vi "Test Read Day Entries DST.vi"(8 "error in (no error)":errorcluster, 10 "Work Folder":path, 11 "Test Data Folder":path) -> (0 "error out":errorcluster, 2 "Report":string, 3 "Passed":bool)   [LabVIEW 2026]
doc: "Checks that Read Day Entries returns the entries of one LOCAL day across the daylight saving changes. The cases assume the PC runs in US Central time (CST/CDT): Sun 8 Mar 2026 is a 23-hour day and Sun 1 Nov 2026 a 25-hour day. Six 30-minute entries are saved with Time Entry Store-INI: A at 23:30 CDT on 8 Mar, B at 00:30 CDT on 9 Mar, C at 23:30 CST on 1 Nov, D at 00:30 CST on 2 Nov, E at 00:30 CDT on 1 Nov and F at 23:30 CST on 7 Mar. Read Day Entries is then called for local noon of 8 Mar, 9 Mar, 1 Nov and 2 Nov: the entry count of each day is checked (1, 1, 2, 1), then that each expected entry ID is among the returned IDs (8 Mar: A, 9 Mar: B, 1 Nov: E and C, 2 Nov: D), independent of order - 9 checks.\n\nInputs: Test Data Folder holds the source copies (Samples); each run works in a new case folder (read-day-dst) under Work Folder. Passed is TRUE when every check passed and no error occurred; Report lists every check.\n\nGenerated by: Claude"
uses:
  Storage/Project Store-INI/Project Store-INI.lvclass
  Storage/Time Entry Store-INI/Time Entry Store-INI.lvclass
  Utilities/Time Management/Time Management.lvlib
  Storage/Time Entry Store/Time Entry Store.lvclass
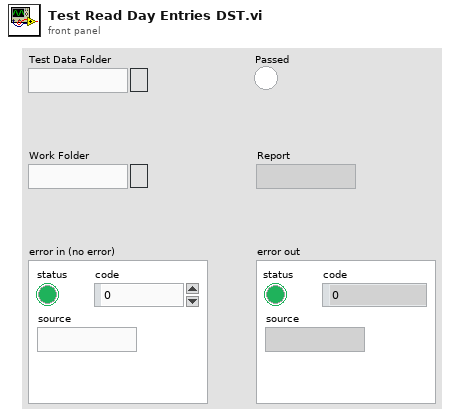
[diagram p1: front panel]
types:
  T1 = cluster{"ID":string, "Project ID":string, "Task ID":string, "Start Time":timestamp, "End Time":timestamp, "Description":string}
  T2 = typedef "Time Entry.ctl" = cluster{"ID":string, "Project ID":string, "Task ID":string, "Start Time":timestamp, "End Time":timestamp, "Description":string}
  T3 = cluster{"ID":string, "Project ID":string, "Task ID":string, "Start Time":timestamp, "End Time":timestamp, "Description":string}[]
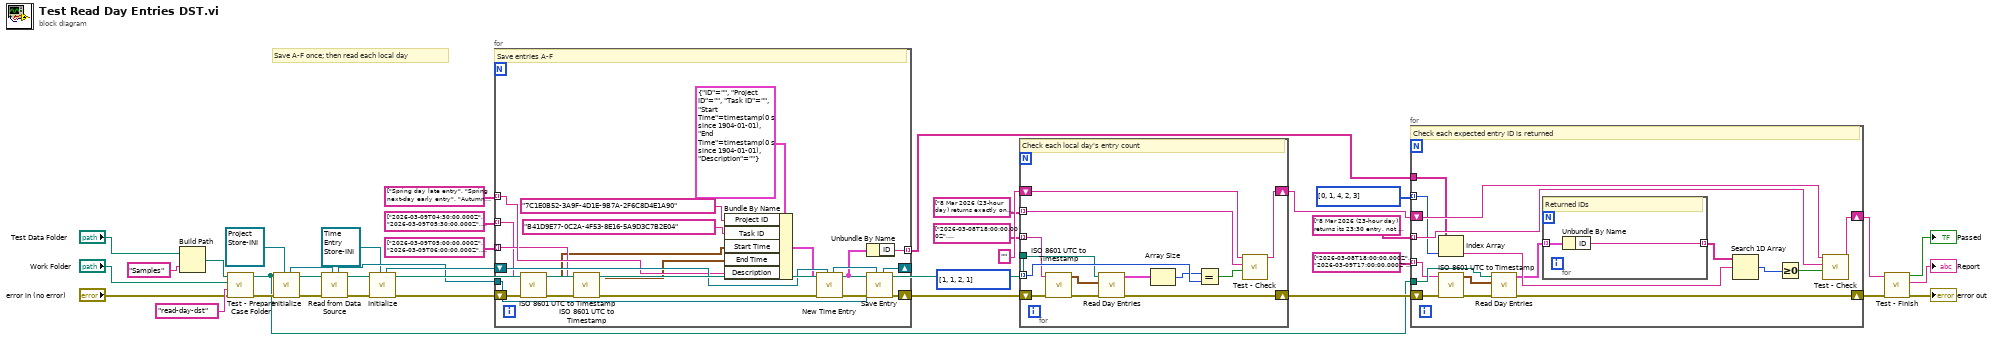
[diagram p0: block diagram]
diagram:
  # "Save A-F once; then read each local day"
  n1 = Build Path(base path="Test Data Folder", name or relative path="Samples" ("Samples")) -> (appended path=w31:path)
  n2 = call "Test - Prepare Case Folder.vi"("error in (no error)"="error in (no error)", "Case Name"="read-day-dst", "Work Folder"="Work Folder", "Source Folder"=w31) -> ("error out"=w32:errorcluster, "Case Folder"=w26:path)  [unwired: 6 in]
  n3 = call-dynamic "Initialize.vi"("Project Store in"=refnum<class "Project Store-INI.lvclass"> refnum ("Project Store-INI"), "error in (no error)"=w32, "Data Folder"=w26) -> ("error out"=w33:errorcluster, "Project Store out"=w34:refnum<class "Project Store-INI.lvclass">)  [unwired: 7 in]
  n4 = call-dynamic "Read from Data Source.vi"("Project Store in"=w34, "error in (no error)"=w33) -> ("error out"=w35:errorcluster, "Project Store out"=w21:refnum<class "Project Store-INI.lvclass">)  [unwired: 8 in]
  n5 = call-dynamic "Initialize.vi"("Time Entry Store in"=refnum<class "Time Entry Store-INI.lvclass"> refnum ("Time Entry Store-INI"), "error in (no error)"=w35, "Data Folder"=w26) -> ("error out"=w23:errorcluster, "Time Entry Store out"=w25:refnum<class "Time Entry Store-INI.lvclass">)  [unwired: 7 in]
  n6 = for {
    tunnel: string[] ["2026-03-09T04:30:00.000Z", "2026-03-09T05:30:00.000Z", "2026-11-02T05:30:00.000Z", "2026-11-02T06:30:00.000Z", "2026-11-01T05:30:00.000Z", "2026-03-08T05:30:00.000Z"] ("Start Times") -> [w42] mode=indexing
    tunnel: string[] ["2026-03-09T05:00:00.000Z", "2026-03-09T06:00:00.000Z", "2026-11-02T06:00:00.000Z", "2026-11-02T07:00:00.000Z", "2026-11-01T06:00:00.000Z", "2026-03-08T06:00:00.000Z"] ("End Times") -> [w45] mode=indexing
    tunnel: string[] ["Spring day late entry", "Spring next-day early entry", "Autumn day late entry", "Autumn next-day early entry", "Autumn day early entry", "Spring previous-day late entry"] ("Descriptions") -> [w47] mode=indexing
    tunnel: w21 -> [w55]
    shift-right: [w53] -> w24
    shift-left: w23 -> [w41]
    shift-right: [w54] -> _
    shift-left: w25 -> [w51]
    tunnel: [w52] -> w22 mode=indexing
    # "Save entries A-F"
    n7 = call "ISO 8601 UTC to Timestamp.vi"("error in (no error)"=w41, "ISO 8601 UTC"=w42) -> ("error out"=w39:errorcluster, "Timestamp"=w40:timestamp)  [unwired: 8 in]
    n8 = call "ISO 8601 UTC to Timestamp.vi"("error in (no error)"=w39, "ISO 8601 UTC"=w45) -> ("error out"=w43:errorcluster, "Timestamp"=w44:timestamp)  [unwired: 8 in]
    n9 = Bundle By Name(cluster=T1 {"ID"="", "Project ID"="", "Task ID"="", "Start Time"=timestamp(0 s since 1904-01-01), "End Time"=timestamp(0 s since 1904-01-01), "Description"=""} ("Time Entry"), "Project ID"="7C1E0B52-3A9F-4D1E-9B7A-2F6C8D4E1A90", "Task ID"="B41D9E77-0C2A-4F53-8E16-5A9D3C7B2E04", "Start Time"=w40, "End Time"=w44, "Description"=w47) -> (w46:T1)
    n10 = call "New Time Entry.vi"("Time Entry Store in"=w51, "error in (no error)"=w43, "Time Entry"=w46) -> ("error out"=w48:errorcluster, "New Time Entry"=w49:T2, "Time Entry Store out"=w50:refnum<class "Time Entry Store-INI.lvclass">)  [unwired: 6 in]
    n11 = Unbundle By Name(w49) -> ("ID"=w52:string)
    n12 = call-dynamic "Save Entry.vi"("Time Entry Store in"=w50, "error in (no error)"=w48, "Project Store"=w55, "Time Entry"=w49) -> ("error out"=w53:errorcluster, "Time Entry Store out"=w54:refnum<class "Time Entry Store-INI.lvclass">)  [unwired: 6 in]
  }
  n13 = for {
    tunnel: string[] ["2026-03-08T18:00:00.000Z", "2026-03-09T17:00:00.000Z", "2026-11-01T18:00:00.000Z", "2026-11-02T18:00:00.000Z"] ("Dates") -> [w59] mode=indexing
    tunnel: string[] ["8 Mar 2026 (23-hour day) returns exactly one entry", "9 Mar 2026 returns exactly one entry", "1 Nov 2026 (25-hour day) returns 2 entries", "2 Nov 2026 returns exactly one entry"] ("Count Check Names") -> [w67] mode=indexing
    tunnel: i32[] [1, 1, 2, 1] ("Expected Counts") -> [w65] mode=indexing
    shift-right: [w66] -> w27
    shift-left: "" ("Report in") -> [w68]
    tunnel: w26 -> [w62]
    shift-right: [w60] -> w28
    shift-left: w24 -> [w58]
    # "Check each local day's entry count"
    n14 = call "ISO 8601 UTC to Timestamp.vi"("error in (no error)"=w58, "ISO 8601 UTC"=w59) -> ("error out"=w56:errorcluster, "Timestamp"=w57:timestamp)  [unwired: 8 in]
    n15 = call "Read Day Entries.vi"("error in (no error)"=w56, "Date"=w57, "Data Folder"=w62) -> ("error out"=w60:errorcluster, "Time Entries"=w61:T3)  [unwired: 7 in]
    n16 = Array Size(array=w61) -> (size(s)=w63:i32)
    n17 = Equal?(x=w63, y=w65) -> (x = y?=w64:bool)
    n18 = call "Test - Check.vi"("Condition"=w64, "Check Name"=w67, "Report in"=w68) -> ("Report out"=w66:string)  [unwired: 7 in, 1 out]
  }
  n19 = for {
    tunnel: string[] ["2026-03-08T18:00:00.000Z", "2026-03-09T17:00:00.000Z", "2026-11-01T18:00:00.000Z", "2026-11-01T18:00:00.000Z", "2026-11-02T18:00:00.000Z"] ("ID Check Dates") -> [w72] mode=indexing
    tunnel: string[] ["8 Mar 2026 (23-hour day) returns its 23:30 entry, not 7 Mar 23:30 or 9 Mar 00:30", "9 Mar 2026 returns its 00:30 entry", "1 Nov 2026 (25-hour day) includes its 00:30 entry", "1 Nov 2026 (25-hour day) includes its 23:30 entry", "2 Nov 2026 returns its 00:30 entry and not the 1 Nov 23:30 entry"] ("ID Check Names") -> [w83] mode=indexing
    tunnel: i32[] [0, 1, 4, 2, 3] ("Expected Entries") -> [w79] mode=indexing
    shift-right: [w82] -> w29
    shift-left: w27 -> [w84]
    tunnel: w26 -> [w75]
    shift-right: [w73] -> w30
    shift-left: w28 -> [w71]
    tunnel: w22 -> [w78]
    # "Check each expected entry ID is returned"
    n20 = Index Array(array=w78, index=w79) -> (element=w77:string)
    n21 = call "ISO 8601 UTC to Timestamp.vi"("error in (no error)"=w71, "ISO 8601 UTC"=w72) -> ("error out"=w69:errorcluster, "Timestamp"=w70:timestamp)  [unwired: 8 in]
    n22 = call "Read Day Entries.vi"("error in (no error)"=w69, "Date"=w70, "Data Folder"=w75) -> ("error out"=w73:errorcluster, "Time Entries"=w74:T3)  [unwired: 7 in]
    n23 = for {
      tunnel: w74 -> [w86] mode=indexing
      tunnel: [w85] -> w76 mode=indexing
      # "Returned IDs"
      n24 = Unbundle By Name(w86) -> ("ID"=w85:string)
    }
    n25 = Search 1D Array(1D array=w76, element=w77) -> (index of element=w80:i32)  [unwired: 1 in]
    n26 = Greater Or Equal To 0?(x=w80) -> (x >= 0?=w81:bool)
    n27 = call "Test - Check.vi"("Condition"=w81, "Check Name"=w83, "Report in"=w84) -> ("Report out"=w82:string)  [unwired: 7 in, 1 out]
  }
  n28 = call "Test - Finish.vi"("error in (no error)"=w30, "Report"=w29) -> ("error out"=→"error out":errorcluster, "Report out"=→"Report":string, "Passed"=→"Passed":bool)  [unwired: 7 in]
